vi "Read from Hardware.vi"(8 "error in (no error)":errorcluster, 10 "Values in":dbl[](array[numeric]), 11 "Rx Execution Unit Implementation in":refnum<class "Rx Execution Unit.lvclass">) -> (0 "error out":errorcluster, 2 "Values out":dbl[](array[numeric]), 3 "Rx Execution Unit Implementation out":refnum<class "Rx Execution Unit.lvclass">)   [LabVIEW 2020, in "AIM ARINC 429 Engine.lvlib" / "Implementation.lvlib" / "Rx Execution Unit.lvclass"]
uses:
  Rx Execution Unit.lvclass
  Execution Unit/Execution Unit.lvclass
  Hardware API/AIM ARINC 429 Hardware API.lvlib
  Custom Device/Custom Device.lvlib
  C:/Users/nitest/Desktop/Git 2020/niveristand-aim-arinc429-custom-device/Source/Custom Device Support/Engine/Implementation/Execution Unit/Execution Unit.lvclass
  C:/Users/nitest/Desktop/Git 2020/niveristand-aim-arinc429-custom-device/Source/Custom Device Support/Engine/Interfaces/Execution Unit/Execution Unit.lvclass
  C:/Users/nitest/Desktop/Git 2020/niveristand-aim-arinc429-custom-device/Source/Custom Device Support/Engine/Implementation/Rx Execution Unit/Rx Execution Unit.lvclass
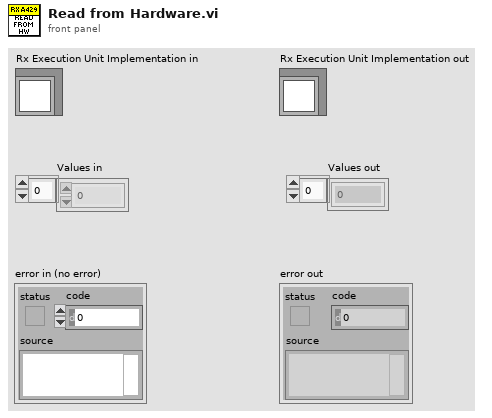
[diagram p1: front panel]
types:
  T1 = typedef "RT Hardware Channel Settings.ctl" = cluster{"channel #":u16, "channel handle":u64, "labels settings for RT":T2[], "speed":T10}
  T2 = typedef "RT Label Settings.ctl" = cluster{"Name":string, "xmlName":string, "label":T3, "transfer period":u32, "SDI_Enabled":bool, "SDI":u8, "parameter driver data":T4, "transfer type":T8, "has timestamp?":bool, "Label Disable/Trigger Channel Reference":T7, "Message Handle":u64, "Initialized?":bool, "Word Initial Raw Value":u32, "Label Timestamp Channel Data Reference":T9, "disabled":bool, "modified":bool}
  T3 = typedef "Label.ctl" = u8
  T4 = typedef "RT Parameters.ctl" = cluster{"parameter definitions":T5[], "Tx parameter refs":T7[]}
  T5 = typedef "Parameter Definition.ctl" = cluster{"start index":i32, "size":i32, "encoding":T6, "signed":bool, "scale multiplier":dbl, "scale offset":dbl, "default value":dbl}
  T6 = typedef "Encoding and Decoding.lvlib/Encoding.ctl" = enum16{"BNR", "BCD", "Discrete"}
  T7 = typedef "Custom Device API.lvlib/Custom Device Item Ref.ctl" = u64
  T8 = typedef "Transfer Type.ctl" = enum16{"Scheduled", "Acyclic", "Block", "Strobe"}
  T9 = typedef "Custom Device API.lvlib/Data Reference.ctl" = i32
  T10 = typedef "Transfer Speed.ctl" = enum16{"LO (12.5 kb/s)", "HI (100 kb/s)"}
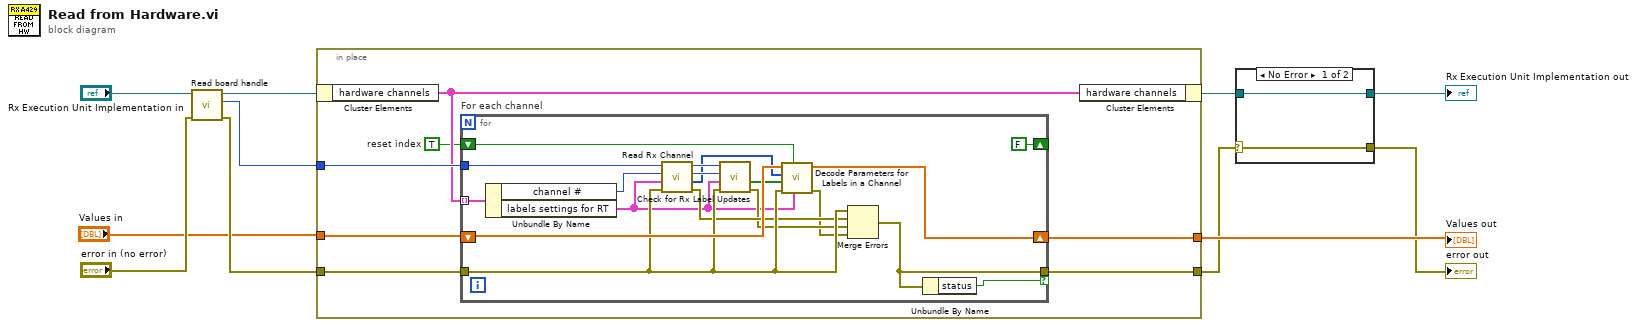
[diagram p0: block diagram]
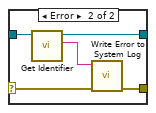
[diagram p2: hidden frame]
diagram:
  n1 = call "Read board handle.vi"("error in (no error)"="error in (no error)", "Execution Unit in"="Rx Execution Unit Implementation in") -> ("error out"=w8:errorcluster, "board handle"=w9:u8, "Execution Unit out"=w10:refnum<class "Rx Execution Unit.lvclass">)  [unwired: 7 in]
  n2 = in-place {
    in-place-border: w9 -> [w18]
    in-place-border: w8 -> [w17]
    in-place-border: [w15] -> w2
    in-place-border: "Values in" -> [w13]
    in-place-border: [w14] -> w5
    w12 = TRUE  # reset index
    n3 = in-place-cluster #1(w10) -> ("hardware channels"=w16:T1[])
    n4 = for "For each channel" {
      tunnel: w18 -> [w34]
      tunnel: w16 -> [w36] mode=indexing
      shift-right: [w33] -> w14
      shift-left: w13 -> [w32]
      shift-right: [FALSE ("reset")] -> _
      shift-left: w12 -> [w31]
      tunnel: w17 -> [w24]
      tunnel: [w20] -> w15 if=w25
      n5 = Unbundle By Name(w36) -> ("channel #"=w35:u16, "labels settings for RT"=w19:T2[])
      n6 = call "Read Rx Channel.vi"("error in"=w24, "labels settings for RT"=w19, "channel number in"=w35, "board handle in"=w34) -> ("error out"=w23:errorcluster, "data out"=w27:u32[], "channel number out"=w28:u8, "board handle out"=w29:u8)  [unwired: 4 in]
      n7 = call "Check for Rx Label Updates.vi"("error in"=w24, "labels settings for RT"=w19, "channel number in"=w28, "board handle in"=w29) -> ("error out"=w22:errorcluster, "labels updated?"=w26:bool[])  [unwired: 4 in, 2 out]
      n8 = call "Decode Parameters for Labels in a Channel.vi"("labels settings for RT"=w19, "reset index"=w31, "error in (no error)"=w24, "updated labels?"=w26, "data words in"=w27, "Parameter Values in"=w32) -> ("error out"=w21:errorcluster, "Parameter Values out"=w33:dbl[])  [unwired: 4 in]
      n9 = Merge Errors(w24, w23, w22, w21) -> (w20:errorcluster)
      n10 = Unbundle By Name(w20) -> ("status"=w25:bool)
    }
    n11 = in-place-cluster #1("hardware channels"=w16) -> (w4:refnum<class "Rx Execution Unit.lvclass">)
  }
  "Values out" <- w5
  n12 = case shown="No Error" w2 {
    selector: w2 -> [w38 w40]
    tunnel: w4 -> [w37 w43]
    tunnel: [w37 w42] -> w3
    tunnel: [w38 w39] -> w1
    frame No Error {
    }
    frame Error {
      n13 = call-dynamic "Get Identifier.vi"("Execution Unit Implementation in"=w43) -> ("Identifier"=w41:string, "Execution Unit Implementation out"=w42:refnum<class "Rx Execution Unit.lvclass">)  [unwired: 8 in, 1 out]
      n14 = call "Write Error to System Log.vi"("error in"=w40, "identifier"=w41) -> ("error out"=w39:errorcluster)  [unwired: 9 in]
    }
  }
  "error out" <- w1
  "Rx Execution Unit Implementation out" <- w3
